vi "Calculate XY.vi"(8 "Delta t":dbl, 9 "Last Length":dbl, 10 "Last High Pressure":dbl, 11 "Acquired Data":dbl[](array[numeric])) -> (0 "Rate/Force":cluster{dbl, dbl}, 1 "delP/Flow":cluster{dbl, dbl}, 2 "Last Length out":dbl, 3 "Last High Pressure out":dbl)   [LabVIEW 2025, in "F18 Blowdown.lvlib" / "F18 Blowdown.lvclass"]
uses:
  F18 Blowdown.lvclass
panel:
  in  "Parameters":T1={"CIS/GPM"=3.85, "AREA ATT'N"=24.2, "AREA RAM"=4.8852, "Beta"=250000.0, "Length"=24.0}
  # "Not be changable"
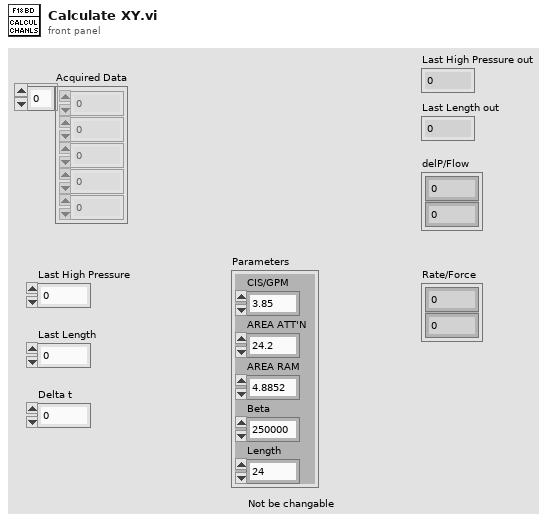
[diagram p1: front panel]
types:
  T1 = cluster{"CIS/GPM":dbl, "AREA ATT'N":dbl, "AREA RAM":dbl, "Beta":dbl, "Length":dbl}
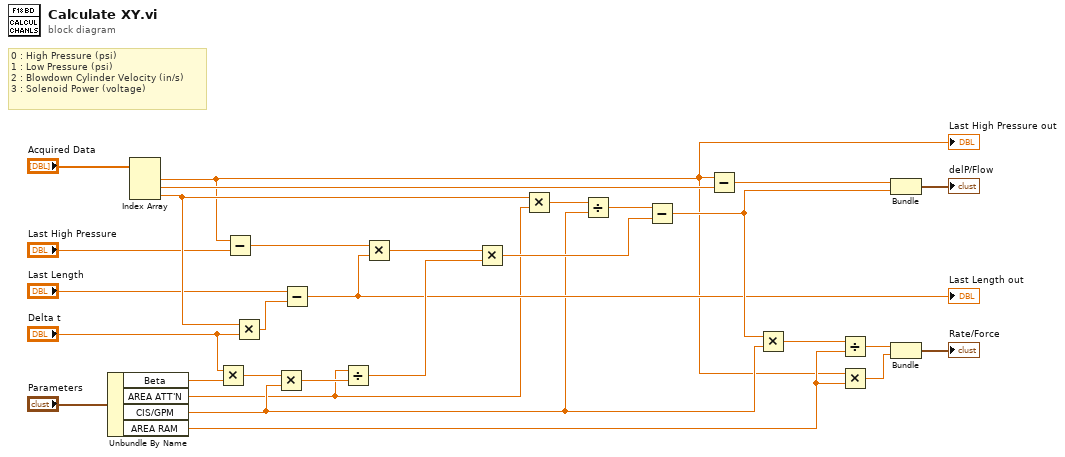
[diagram p0: block diagram]
diagram:
  # "0 : High Pressure (psi)\n1 : Low Pressure (psi)\n2 : Blowdown Cylinder Velocity (in/s)\n3 : Solenoid Power (voltage)"
  n1 = Unbundle By Name("Parameters") -> ("Beta"=w9:dbl, "AREA ATT'N"=w2:dbl, "CIS/GPM"=w3:dbl, "AREA RAM"=w17:dbl)
  n2 = Index Array(array="Acquired Data") -> (element #1=w1:dbl, element #2=w19:dbl, element #3=w20:dbl)  [unwired: 3 in]
  "Last High Pressure out" <- w1
  n3 = Multiply(x="Delta t", y=w9) -> (x*y=w18:dbl)
  n4 = Subtract(x=w1, y="Last High Pressure") -> (x-y=w28:dbl)
  n5 = Multiply(x=w20, y="Delta t") -> (x*y=w25:dbl)
  n6 = Multiply(x=w18, y=w3) -> (x*y=w29:dbl)
  n7 = Subtract(x="Last Length", y=w25) -> (x-y=w4:dbl)
  "Last Length out" <- w4
  n8 = Divide(x=w2, y=w29) -> (x/y=w26:dbl)
  n9 = Multiply(x=w28, y=w4) -> (x*y=w27:dbl)
  n10 = Multiply(x=w27, y=w26) -> (x*y=w22:dbl)
  n11 = Multiply(x=w20, y=w2) -> (x*y=w24:dbl)
  n12 = Divide(x=w24, y=w3) -> (x/y=w23:dbl)
  n13 = Subtract(x=w23, y=w22) -> (x-y=w15:dbl)
  n14 = Subtract(x=w1, y=w19) -> (x-y=w16:dbl)
  n15 = Multiply(x=w15, y=w3) -> (x*y=w21:dbl)
  n16 = Divide(x=w21, y=w17) -> (x/y=w13:dbl)
  n17 = Multiply(x=w1, y=w17) -> (x*y=w12:dbl)
  n18 = Bundle(w16, w15) -> (→"delP/Flow":cluster{dbl, dbl})  [unwired: 1 in]
  n19 = Bundle(w13, w12) -> (→"Rate/Force":cluster{dbl, dbl})  [unwired: 1 in]
